vi "Example - Publish to localhost.vi"() -> ()   [LabVIEW 2019]
uses:
  src/KoRE-MQTT.lvlib
  src/KoRE-MQTT/Public/TypeDefs/MQTT Version.ctl
panel:
  in  "QoS 3":T1(ring)
  in  "Port":u16=1883
  in  "Host":string="localhost"
  in  "Password":string
  in  "Username":string
  in  "Version":T2=4 items=["3.11"=4, "5.0"=5]
  out "Messages / Second":dbl
  out "Variant":variant
  out "Total Messages":i32
  in  "Num vars":i32=500 min=1 max=5000 step=1
  in  "hz":u32=10 min=1 max=100 step=1
  in  "stop":bool
  # "Use this VI to stress test your local broker and to stress test this MQTT library. While you can use this VI to generate a lot of publish packets, you can use the \"Example - MQTT performance test.vi\" to stress test reception of the same published packets."
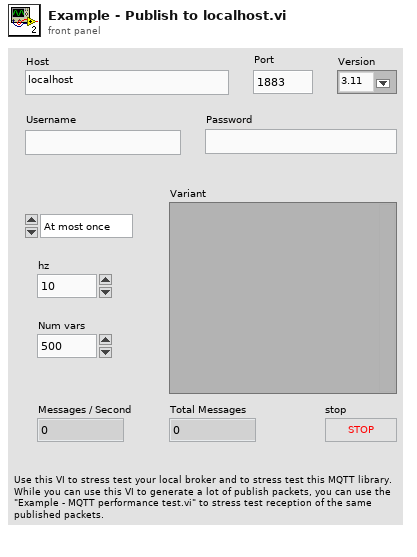
[diagram p1: front panel]
types:
  T1 = enum16{"At most once", "At least once", "Exactly once"}
  T2 = typedef "KoRE-MQTT.lvlib/MQTT Version.ctl" = u8
  T3 = typedef "KoRE-MQTT.lvlib/MQTT Refnum.ctl" = refnum<vi>
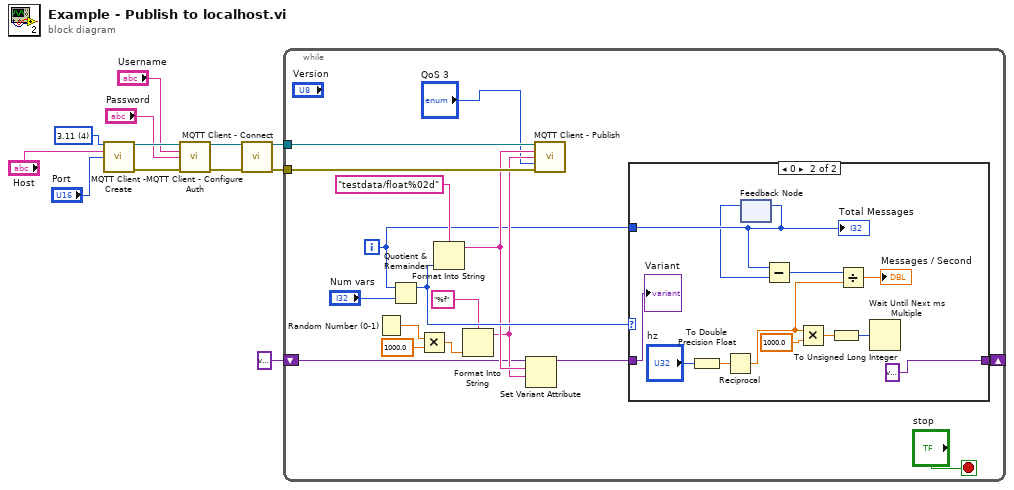
[diagram p0: block diagram]
diagram:
  w10 = T2 4 items=["3.11"=4, "5.0"=5] ("Version (3.11)")
  n1 = call "MQTT Client - Create.vi"("Version (3.11)"=w10, "Host (localhost)"="Host", "Port (1883)"="Port") -> ("MQTT Session"=w8:T3, "error out"=w7:errorcluster)  [unwired: 11 in]
  n2 = call "MQTT Client - Configure Auth.vi"("MQTT Session"=w8, "Client ID"="Username", "Username"="Password", "error in (no error)"=w7) -> ("MQTT Session"=w6:T3, "error out"=w5:errorcluster)  [unwired: 10 in]
  n3 = call "MQTT Client - Connect.vi"("MQTT ref in"=w6, "error in (no error)"=w5) -> ("mqtt ref"=w12:T3, "error out"=w11:errorcluster)  [unwired: 9 in, 3 out]
  n4 = while {
    tunnel: w12 -> [w29]
    tunnel: w11 -> [w28]
    shift-right: [w16] -> _
    shift-left: variant -> [w18]
    i -> [w14]
    stop <- "stop" stop-if-true
    n5 = Random Number (0-1)() -> (number: 0 to 1=w25:dbl)
    n6 = Quotient & Remainder(x=w14, y="Num vars") -> (x-y*floor(x/y)=w21:i32)  [unwired: 1 out]
    n7 = Multiply(x=w25, y=1000.0) -> (x*y=w23:dbl)
    n8 = Format Into String(format string="testdata/float%02d", w21) -> (resulting string=w20:string)  [unwired: 2 in, 1 out]
    n9 = Format Into String(format string="%f", w23) -> (resulting string=w19:string)  [unwired: 2 in, 1 out]
    n10 = Set Variant Attribute(Variant=w18, name=w20, value=w19) -> (Variant out=w17:variant)  [unwired: 1 in, 2 out]
    n11 = call "MQTT Client - Publish.vi"("MQTT Session"=w29, "Topic"=w20, "Message"=w19, "QoS"="QoS 3", "error in"=w28) -> ()  [unwired: 9 in, 2 out]
    n12 = case shown="0" w21 {
      tunnel: w17 -> [w30 w38]
      tunnel: [w30 variant] -> w16
      tunnel: w14 -> [_ w36]
      frame Default {
      }
      frame 0 {
        n13 = To Double Precision Float(number="hz") -> (double precision float=w40:dbl)
        n14 = Reciprocal(x=w40) -> (1/x=w31:dbl)
        n15 = feedback-in #1(w36) -> ()
        n16 = feedback #1() -> (w35:i32)  [unwired: 1 in]
        n17 = Subtract(x=w36, y=w35) -> (x-y=w34:i32)
        n18 = Multiply(x=w31, y=1000.0) -> (x*y=w33:dbl)
        n19 = To Unsigned Long Integer(number=w33) -> (unsigned 32bit integer=w39:u32)
        n20 = Divide(x=w34, y=w31) -> (x/y=→"Messages / Second":dbl)
        n21 = Wait Until Next ms Multiple(millisecond multiple=w39) -> ()  [unwired: 1 out]
        "Variant" <- w38
        "Total Messages" <- w36
      }
    }
  }
